vi "Var - Test variable.vi"(5 "VC Handle":T2=-1, 6 "error in":bool, 9 "name_spec":string) -> (0 "error out":bool, 1 "err code":T1 items=["No error", "Invalid variable type", "Variable not found", "Variable already exists", "Invalid context handle", "Input error", "Invalid data format", "No history attached", "History already attached", "Invalid history parameters", "Wrong variable name", "Wrong alias name", "Non-unique alias", "Alias not found", "No alias associated", "Alias already associated", "Wrong context name", "Non-unique context name", "Context name not found", "Invalid parameter", "Generic error", "Memory Full", "Unrecognized LV error", "Unknown error code"], 2 "type":u32(ring) items=["String", "DBL Number", "identifier", "1D Array of DBL", "2D Array of DBL", "CDB Number", "1D Array of CDB", "2D Array of CDB", "1D Array of String", "2D Array of String", "Unknown data type"], 3 "dup name_spec":string, 4 "dup VC Handle":T2=-1)   [LabVIEW 2021]
doc: "<b>*** DEPRECATED ***</b>\n\nThe VI tests a variable. If the specified variable exists, VI returns its type. See online help for the VI for more information.\n\n<VC Handle> control has to contain a handle of variable context if <name_spec> control contains a variable name. In order to test a global variable, pass -1 to it. <VC Handle> is ignored if <name_spec> refers to a variable by alias.\n\n<name_spec> control has to contain a name specifier referring to a desired variable. Generic format of a name specifier is\n [name][=alias]\n, where\n 'name' is a variable name.\n 'alias' is an alias associated with a variable; it must follow equal sign (=).\nEither 'name' or '=alias' may be omitted but not both.\n\n::: CalcExpress Toolkit :::\nCopyright (c) 2000-2026 Konstantin Shifershteyn. All rights reserved."
uses:
  cetypes.llb/VarMan Variable Context Handle.ctl
  cetypes.llb/VarMan Error Code.ctl
  cersrc/celveng32.dll
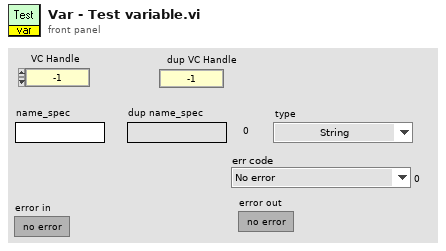
[diagram p1: front panel]
types:
  T1 = typedef "VarMan Error Code.ctl" = u16
  T2 = typedef "VarMan Variable Context Handle.ctl" = i32
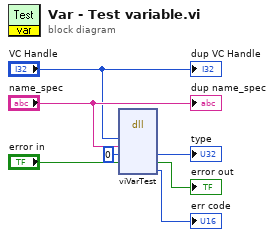
[diagram p0: block diagram]
diagram:
  n1 = dll-call lib="C:/LV Projects/CalcExpress 40 LV2021/vi.lib/addons/CalcExpress/cersrc/celveng*.dll" fn="viVarTest"("vch"="VC Handle", "name"="name_spec", "type"=u32 0, "errf"="error in") -> ("type"=→"type":u32, "errf"=→"error out":bool, "err code"=→"err code":T1)  [unwired: 7 in, 2 out]
  "dup VC Handle" <- "VC Handle"
  "dup name_spec" <- "name_spec"
